vi "Substitute Actor.vi"(10 "Substitute Actor in":refnum<class "Actor.lvclass">, 11 "Current CommonState":refnum<class "CoordinatorState.lvclass">) -> (0 "error out":errorcluster, 2 "Substitute Actor out":refnum<class "Actor.lvclass">)   [LabVIEW 2014, in "States.lvlib" / "CoordinatorState.lvclass"]
doc: "(<B>Filename</B>: Actor Framework.lvlib:Actor.lvclass:Substitute Actor.vi)\n\nThis method copies information from the <b>Current Actor</b> to the <b>Substitute Actor</b>, including the to-self and the to-caller queue references. The purpose of this function is to allow an actor to define a method that replaces itself with another actor, useful for implementing a State Pattern Actor. Child classes should override this method to copy any additional fields that they need from the current to the substitute.\n\nThis method may return error code 678010: Illegal substitution. Overrides of this method may choose to return this error if the new actor is not one that is an appropriate substitute for the current actor, for whatever standards of \"appropriate\" are chosen for the current actor."
uses:
  CoordinatorState.lvclass
  <vilib>/ActorFramework/Actor/Actor.lvclass
  CoordinatorState.lvclass/CoordinatorState.ctl
  <vilib>/NI/Actors/State Actor/State Actor/State Actor.lvclass
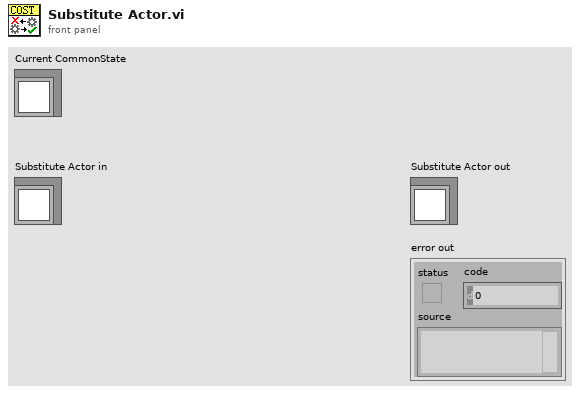
[diagram p1: front panel]
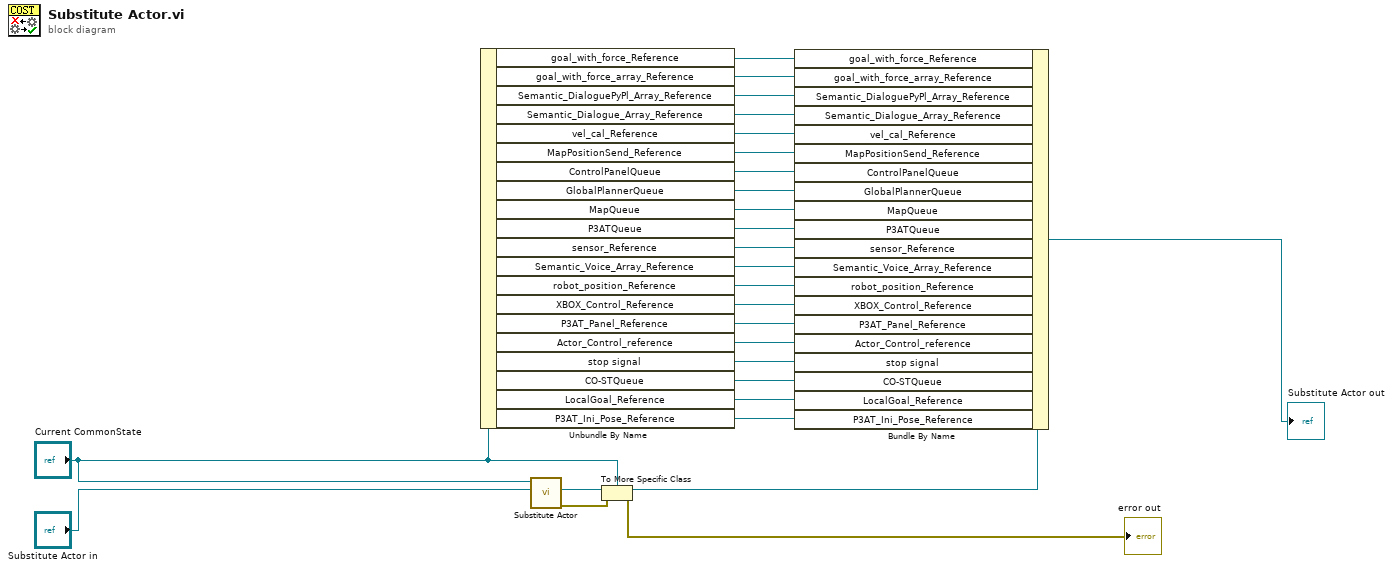
[diagram p0: block diagram]
diagram:
  n1 = Unbundle By Name("Current CommonState") -> ("goal_with_force_Reference"=w2:refnum<vi>, "goal_with_force_array_Reference"=w1:refnum<vi>, "Semantic_DialoguePyPl_Array_Reference"=w3:refnum<vi>, "Semantic_Dialogue_Array_Reference"=w4:refnum<vi>, "vel_cal_Reference"=w5:refnum<vi>, "MapPositionSend_Reference"=w6:refnum<vi>, "ControlPanelQueue"=w19:refnum<class "Message Enqueuer.lvclass">, "GlobalPlannerQueue"=w18:refnum<class "Message Enqueuer.lvclass">, "MapQueue"=w17:refnum<class "Message Enqueuer.lvclass">, "P3ATQueue"=w16:refnum<class "Message Enqueuer.lvclass">, "sensor_Reference"=w15:refnum<vi>, "Semantic_Voice_Array_Reference"=w14:refnum<vi>, "robot_position_Reference"=w13:refnum<vi>, "XBOX_Control_Reference"=w12:refnum<vi>, "P3AT_Panel_Reference"=w11:refnum<vi>, "Actor_Control_reference"=w10:refnum<vi>, "stop signal"=w9:refnum<user-event>, "CO-STQueue"=w8:refnum<class "Message Enqueuer.lvclass">, "LocalGoal_Reference"=w7:refnum<vi>, "P3AT_Ini_Pose_Reference"=w20:refnum<vi>)
  n2 = call-parent "Substitute Actor.vi"("Substitute Actor in"="Substitute Actor in", "Current Actor"="Current CommonState") -> ("error out"=w22:errorcluster, "Substitute Actor out"=w27:refnum<class "Actor.lvclass">)  [unwired: 8 in]
  n3 = To More Specific Class(target class="Current CommonState", reference=w27, error in=w22) -> (specific class reference=w25:refnum<class "CoordinatorState.lvclass">, error out=→"error out":errorcluster)
  n4 = Bundle By Name(cluster=w25, "goal_with_force_Reference"=w2, "goal_with_force_array_Reference"=w1, "Semantic_DialoguePyPl_Array_Reference"=w3, "Semantic_Dialogue_Array_Reference"=w4, "vel_cal_Reference"=w5, "MapPositionSend_Reference"=w6, "ControlPanelQueue"=w19, "GlobalPlannerQueue"=w18, "MapQueue"=w17, "P3ATQueue"=w16, "sensor_Reference"=w15, "Semantic_Voice_Array_Reference"=w14, "robot_position_Reference"=w13, "XBOX_Control_Reference"=w12, "P3AT_Panel_Reference"=w11, "Actor_Control_reference"=w10, "stop signal"=w9, "CO-STQueue"=w8, "LocalGoal_Reference"=w7, "P3AT_Ini_Pose_Reference"=w20) -> (→"Substitute Actor out":refnum<class "CoordinatorState.lvclass">)
